vi "_Rect2TopLeftPoint.vi"(4 "bounds":T1) -> (1 "TopLeft point":cluster{"x":i32, "y":i32})   [LabVIEW 2012]
doc: "Extracts the top left point from the rectangle coordinates (bounds)."
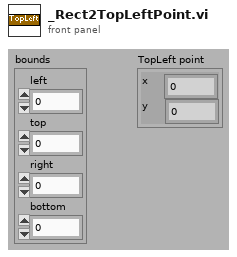
[diagram p1: front panel]
types:
  T1 = cluster{"left":i16, "top":i16, "right":i16, "bottom":i16}
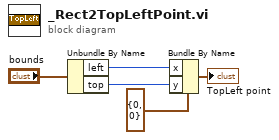
[diagram p0: block diagram]
diagram:
  n1 = Unbundle By Name("bounds") -> ("left"=w2:i16, "top"=w1:i16)
  n2 = Bundle By Name(cluster=cluster{"x":i32, "y":i32} {"x"=0, "y"=0} ("Point"), "x"=w2, "y"=w1) -> (→"TopLeft point":cluster{"x":i32, "y":i32})
